vi "1b.get_system_name_parameters.vi"() -> ()   [LabVIEW 2017]
uses:
  <vilib>/Instr/_visa.llb/VISA Configure Serial Port (Instr).vi
panel:
  out "read buffer 2":string
  out "VISA resource name out":refnum<visa-resource-name>
  out "read buffer":string
  in  "VISA resource name":refnum<visa-resource-name>="COM3" caption="Serial COM port"
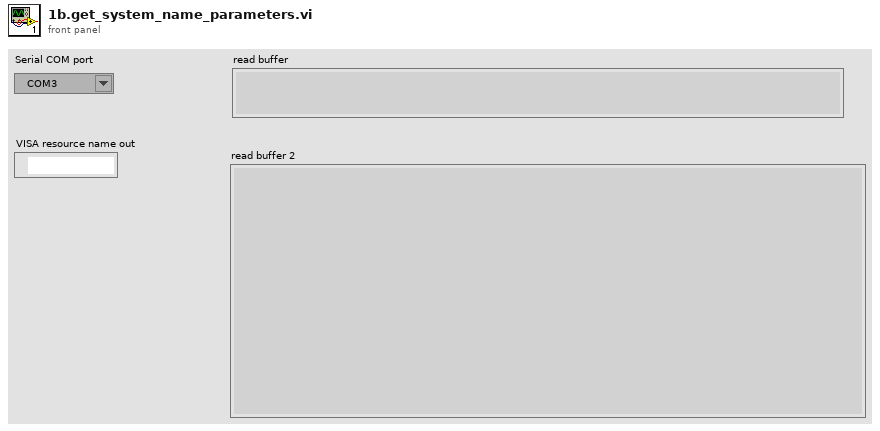
[diagram p1: front panel]
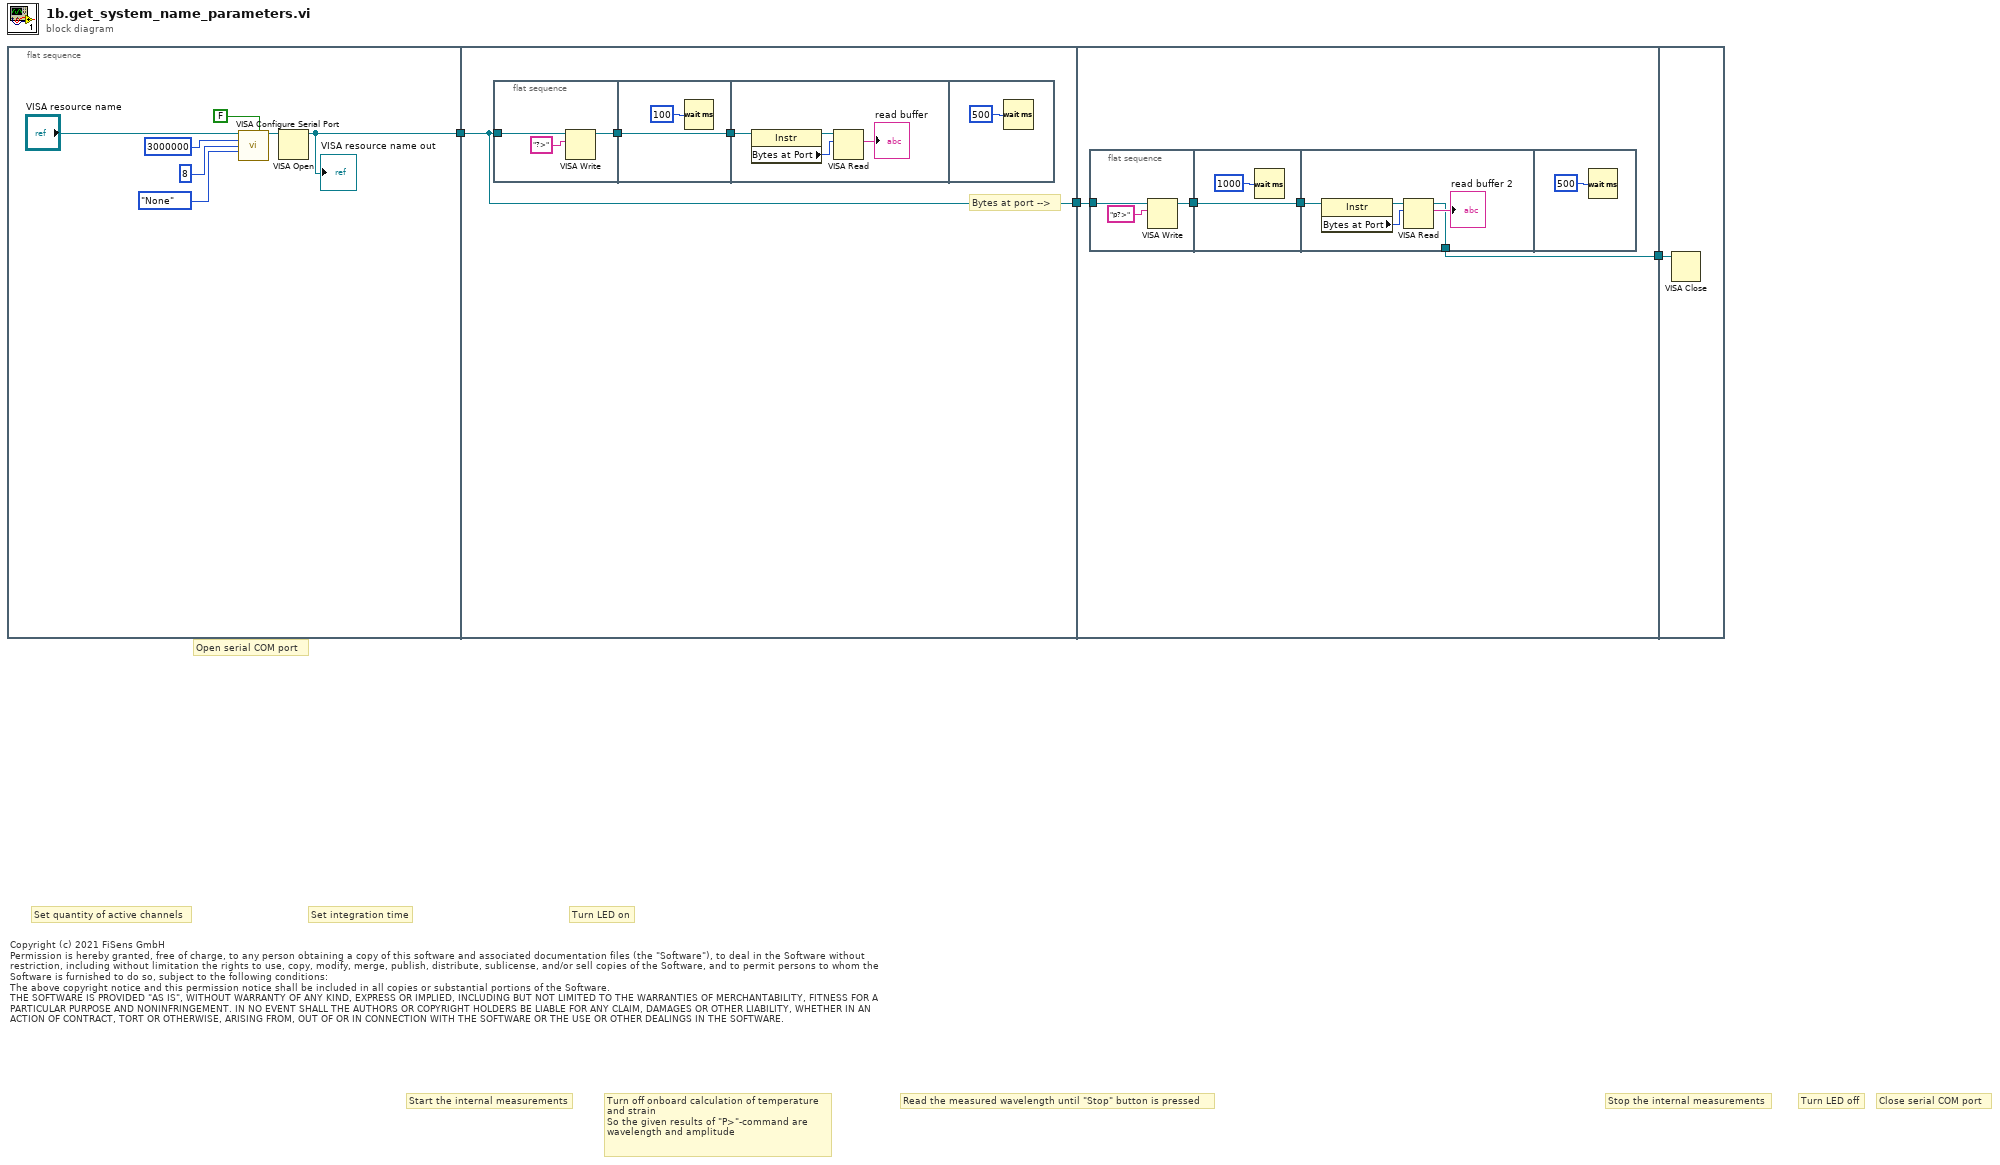
[diagram p0: block diagram]
diagram:
  # "Copyright (c) 2021 FiSens GmbH\nPermission is hereby granted, free of charge, to any person obtaining a copy of this software and associated documentation files (the \"Software\"), to deal in the Software without restriction, including without limitation the rights to use, copy, modify, merge, publish, distribute, sublicense, and/or sell copies of the Software, and to permit persons to whom the Software is furnished to do so, subject to the following conditions:\nThe above copyright notice and this permission notice shall be included in all copies or substantial portions of the Software.\nTHE SOFTWARE IS PROVIDED \"AS IS\", WITHOUT WARRANTY OF ANY KIND, EXPRESS OR IMPLIED, INCLUDING BUT NOT LIMITED TO THE WARRANTIES OF MERCHANTABILITY, FITNESS FOR A PARTICULAR PURPOSE AND NONINFRINGEMENT. IN NO EVENT SHALL THE AUTHORS OR COPYRIGHT HOLDERS BE LIABLE FOR ANY CLAIM, DAMAGES OR OTHER LIABILITY, WHETHER IN AN ACTION OF CONTRACT, TORT OR OTHERWISE, ARISING FROM, OUT OF OR IN CONNECTION WITH THE SOFTWARE OR THE USE OR OTHER DEALINGS IN THE SOFTWARE."
  # "Turn off onboard calculation of temperature and strain\nSo the given results of \"P>\"-command are wavelength and amplitude"
  # "Close serial COM port"
  # "Turn LED off"
  # "Stop the internal measurements"
  # "Read the measured wavelength until \"Stop\" button is pressed"
  # "Start the internal measurements"
  # "Turn LED on"
  # "Set integration time"
  # "Open serial COM port"
  # "Set quantity of active channels"
  n1 = flat-sequence {
    tunnel: [w6] -> w3
    tunnel: w3 -> [w11]
    tunnel: [w11] -> w2
    tunnel: w2 -> [w25]
    tunnel: [w24] -> w1
    tunnel: w1 -> [w39]
    frame #0 {
      n2 = call-poly "VISA Configure Serial Port"("VISA resource name"="VISA resource name", "Enable Termination\nChar (T)"=FALSE ("Enable Termination\nChar (T)"), "baud rate (9600)"=u32 3000000, "data bits (8)"=u16 8, "parity (0:none)"=enum16{"None", "Odd", "Even", "Mark", "Space"}."None") -> ("VISA resource name out"=w10:refnum<visa-resource-name>)  [unwired: 9 in, 1 out]
      n3 = VISA Open(VISA resource name=w10) -> (VISA resource name=w6:refnum<visa-resource-name>)  [unwired: 4 in, 1 out]
      "VISA resource name out" <- w6
    }
    frame #1 {
      # "Bytes at port -->"
      n4 = flat-sequence {
        tunnel: [w16] -> w13
        tunnel: w11 -> [w15]
        tunnel: [w17] -> w12
        tunnel: w13 -> [w17]
        tunnel: w12 -> [w22]
        frame #0 {
          n5 = VISA Write(VISA resource name=w15, write buffer="?>") -> (VISA resource name out=w16:refnum<visa-resource-name>)  [unwired: 1 in, 2 out]
        }
        frame #1 {
          n6 = Wait (ms)(milliseconds to wait=u32 100 ("Zu wartende ms")) -> ()  [unwired: 1 out]
        }
        frame #2 {
          n7 = property class="Instr"(reference=w22) -> (reference out=w21:refnum<visa-resource-name>, "Bytes at Port"=w20:u32)  [unwired: 1 in, 1 out]
          n8 = VISA Read(VISA resource name=w21, byte count=w20) -> (read buffer=→"read buffer":string)  [unwired: 1 in, 3 out]
        }
        frame #3 {
          n9 = Wait (ms)(milliseconds to wait=u32 500 ("Zu wartende ms")) -> ()  [unwired: 1 out]
        }
      }
    }
    frame #2 {
      n10 = flat-sequence {
        tunnel: [w30] -> w27
        tunnel: w25 -> [w28]
        tunnel: [w31] -> w26
        tunnel: w27 -> [w31]
        tunnel: w26 -> [w37]
        tunnel: [w33] -> w24
        frame #0 {
          n11 = VISA Write(VISA resource name=w28, write buffer="p?>") -> (VISA resource name out=w30:refnum<visa-resource-name>)  [unwired: 1 in, 2 out]
        }
        frame #1 {
          n12 = Wait (ms)(milliseconds to wait=u32 1000 ("Zu wartende ms")) -> ()  [unwired: 1 out]
        }
        frame #2 {
          n13 = property class="Instr"(reference=w37) -> (reference out=w36:refnum<visa-resource-name>, "Bytes at Port"=w35:u32)  [unwired: 1 in, 1 out]
          n14 = VISA Read(VISA resource name=w36, byte count=w35) -> (VISA resource name out=w33:refnum<visa-resource-name>, read buffer=→"read buffer 2":string)  [unwired: 1 in, 2 out]
        }
        frame #3 {
          n15 = Wait (ms)(milliseconds to wait=u32 500 ("Zu wartende ms")) -> ()  [unwired: 1 out]
        }
      }
    }
    frame #3 {
      n16 = VISA Close(VISA resource name=w39) -> ()  [unwired: 1 in, 1 out]
    }
  }
